vi "demo_proj.vi"() -> ()   [LabVIEW 2015]
doc: "该模板用于创建生产者／消费者模式的应用程序，以事件驱动的方式，生成队列中的项。如需通过响应事件实现代码的异步执行，同时不影响用户界面的响应速度，可考虑用该模式替代用户界面事件处理器模式。"
panel:
  in  "设备类型":enum16{"LAN", "USB"}(ring)=enum."USB"
  in  "波形分析":bool
  in  "读取波形":bool
  in  "波形读取模式":enum32{"bin", "csv"}(radio)
  in  "读取的字节数":u32=400
  in  "读数据":bool
  in  "发指令":bool
  in  "指令集合":string(combo)="mea:all?;"
  in  "清空信息":bool
  out "输出信息":string
  in  "关闭设备":bool
  in  "超时时间(ms)":u32=2000
  out "会话ID":i32
  in  "打开设备":bool
  in  "设备集合":string(combo)
  in  "搜索设备":bool caption="元素入队列"
  in  "停止":bool
  out "数据缓存":u8[](array[numeric])
  out "波形图":sgl[](graph)
  out "波形数据":sgl[](array[numeric])
  out "csv文件输出路径":string
  out "data_out":sgl[](array[numeric])
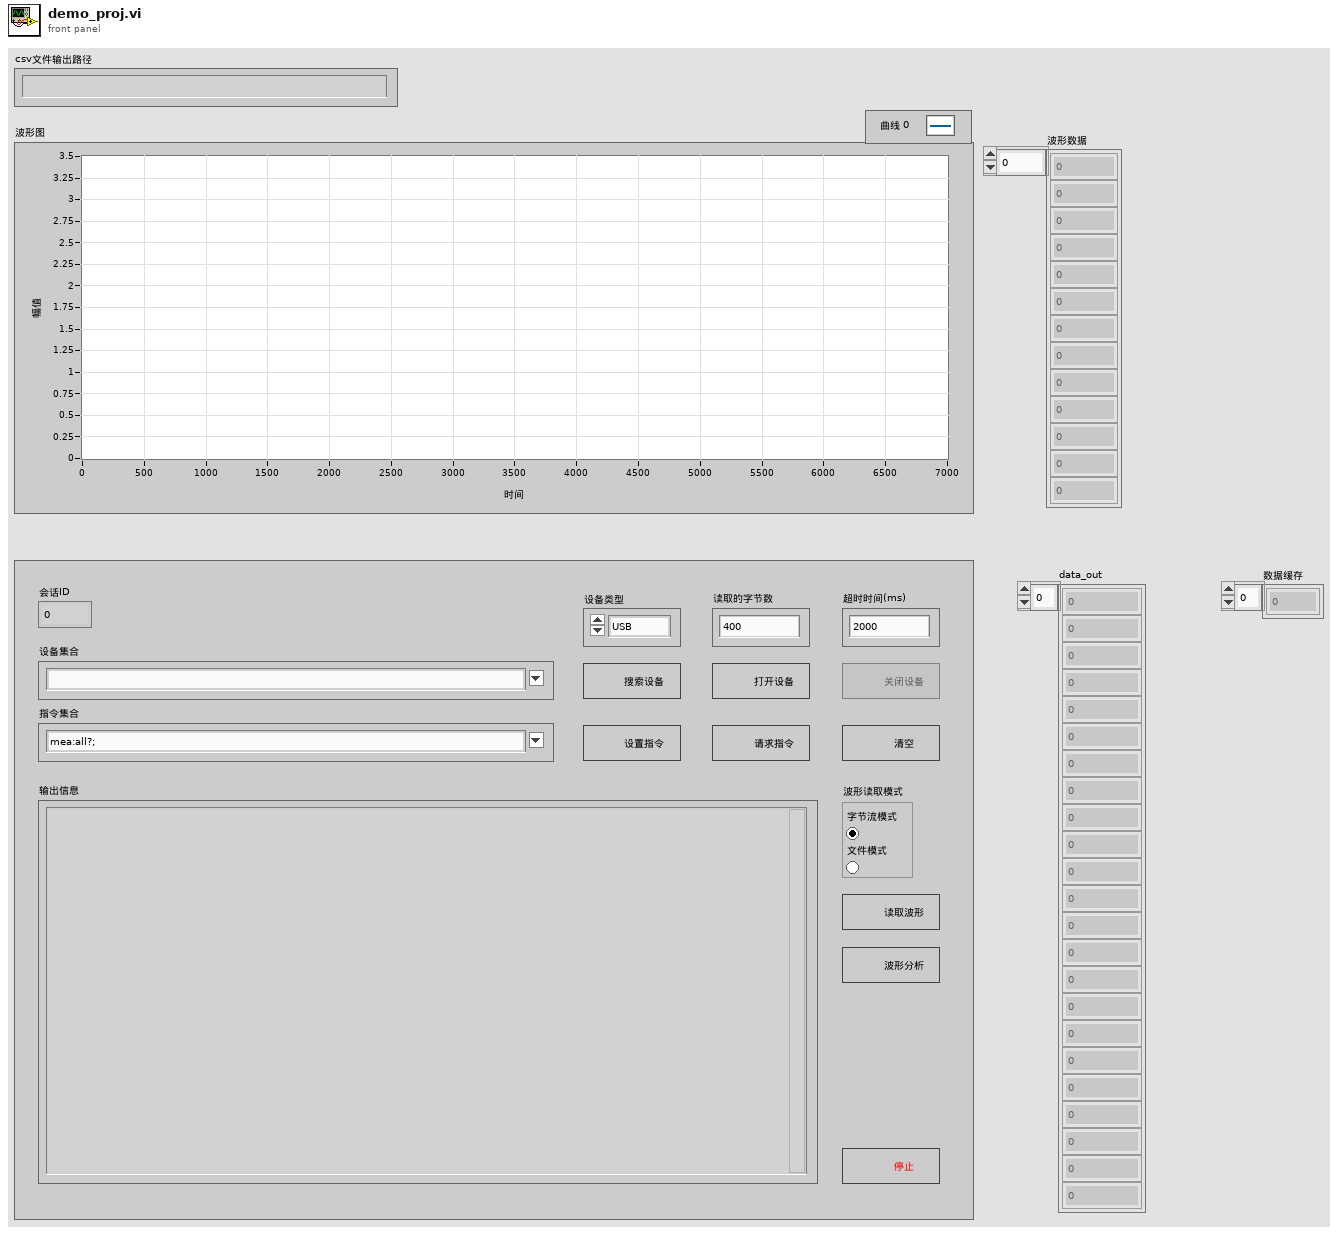
[diagram p1: front panel]
types:
  T1 = enum8{"Enabled", "Disabled", "Disabled and Grayed Out"}
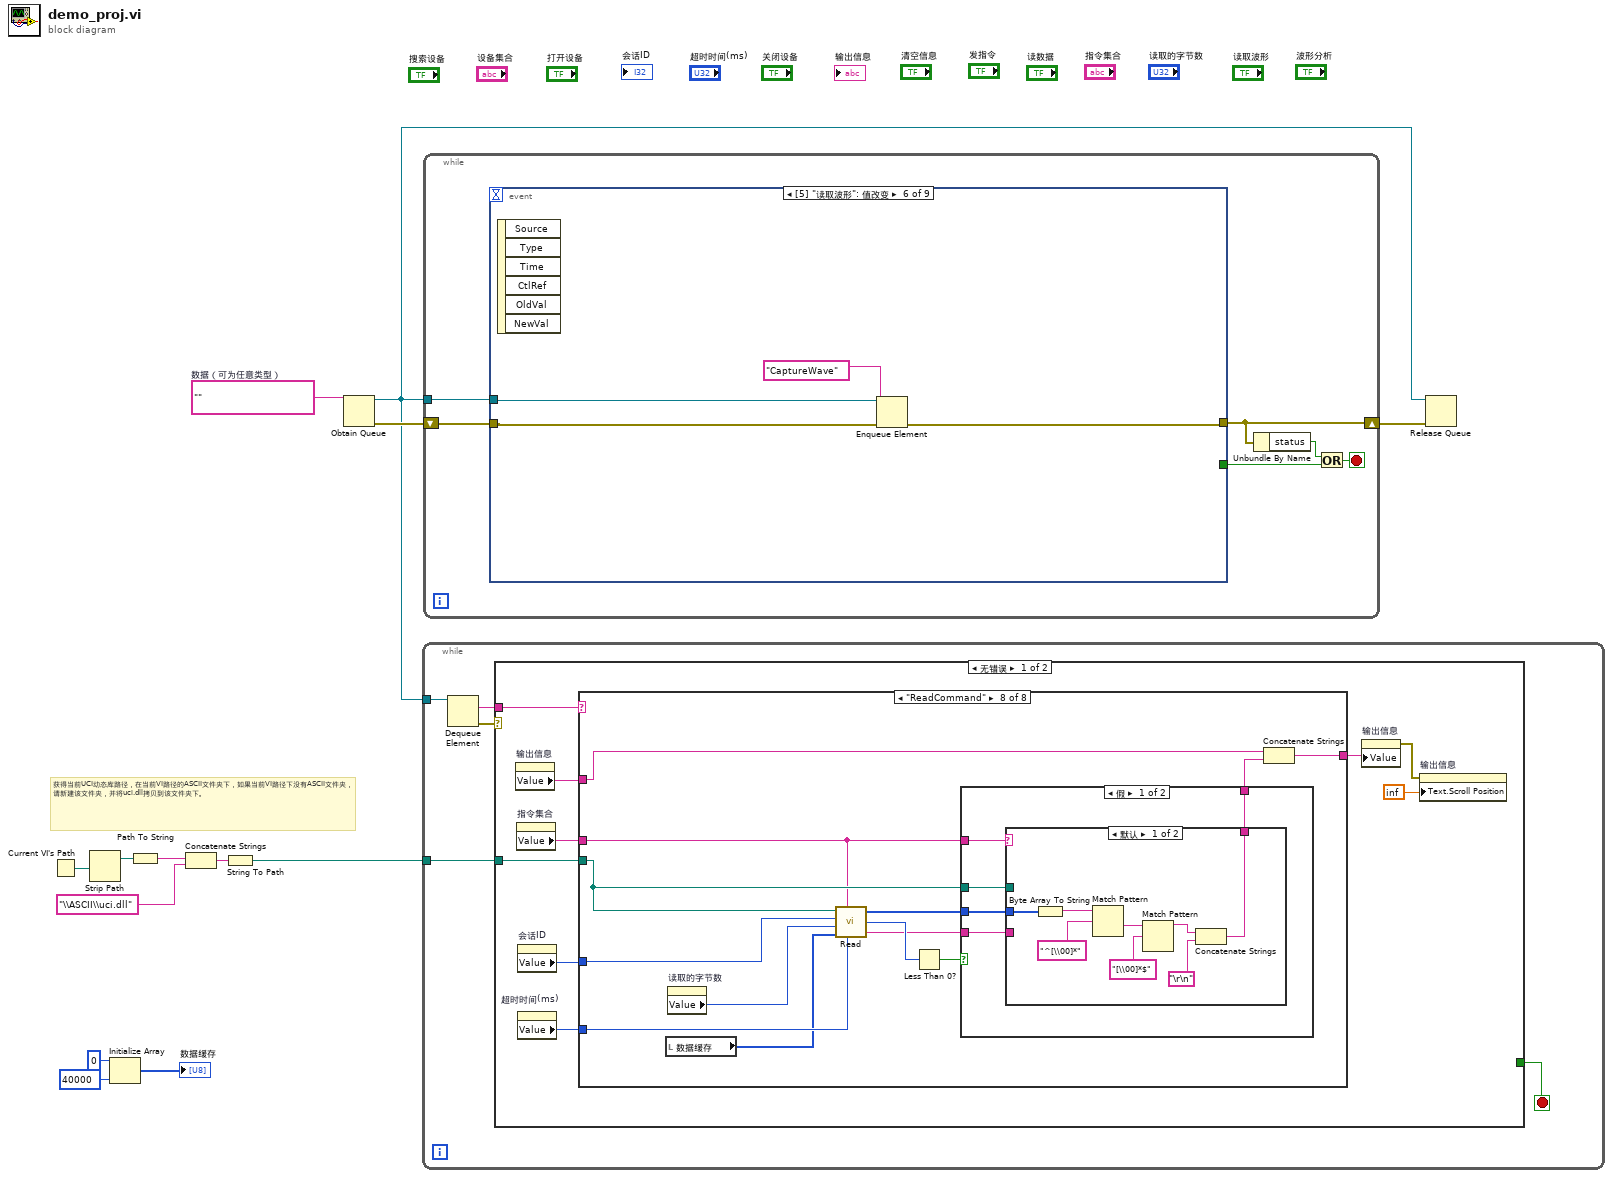
[diagram p0: block diagram]
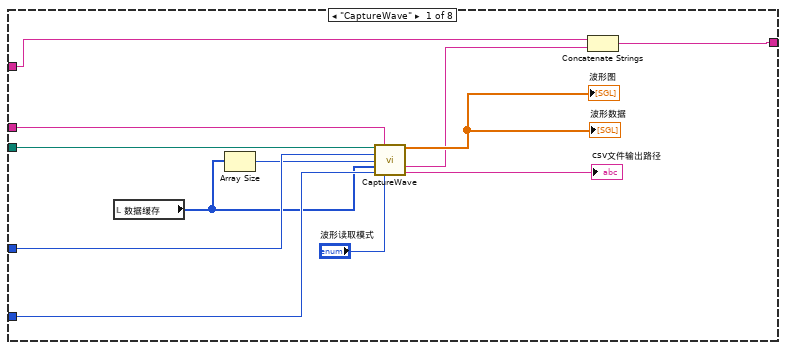
[diagram p2: hidden frame]
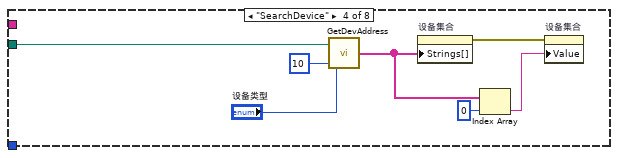
[diagram p5: hidden frame]
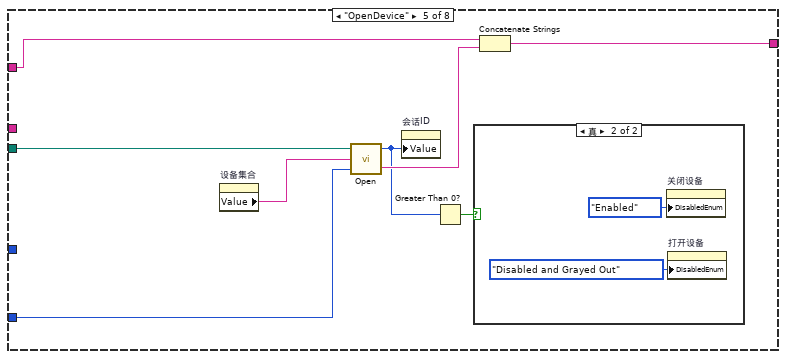
[diagram p6: hidden frame]
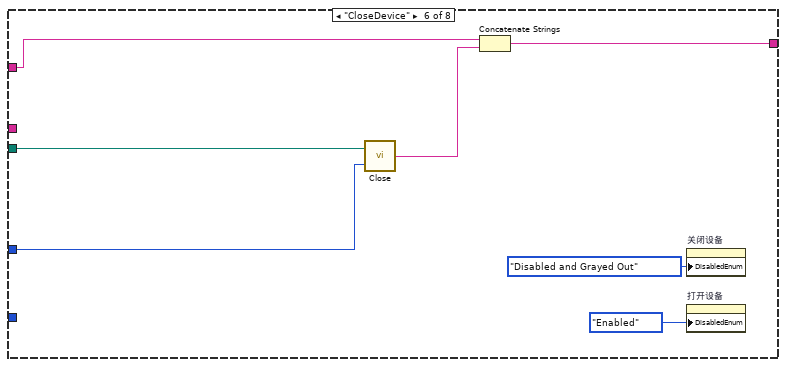
[diagram p8: hidden frame]
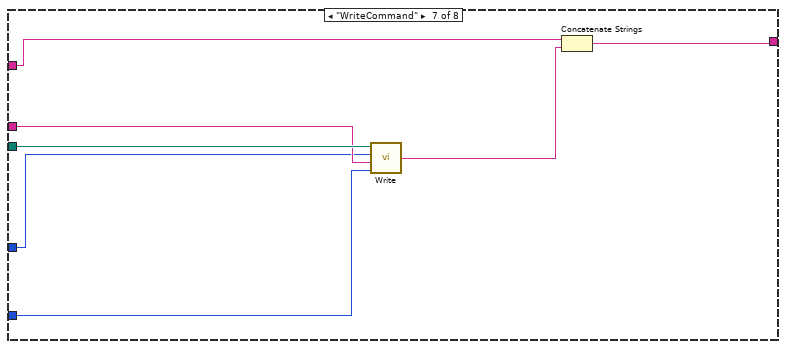
[diagram p9: hidden frame]
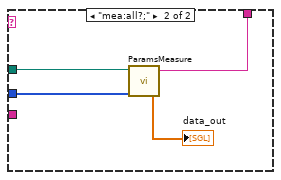
[diagram p10: hidden frame]
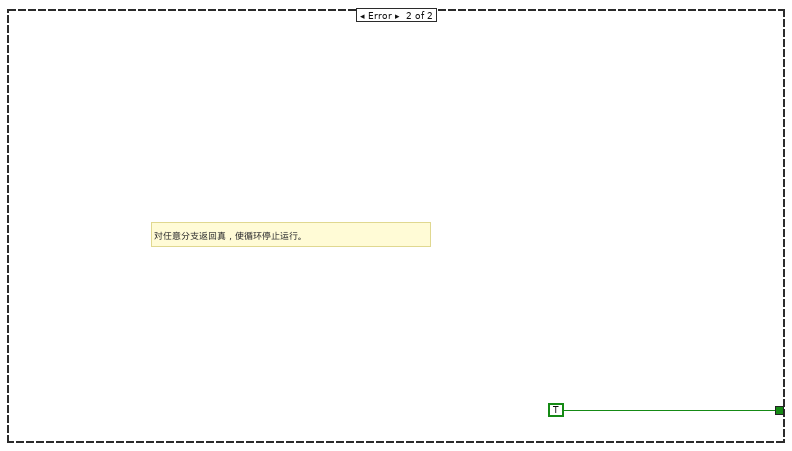
[diagram p12: hidden frame]
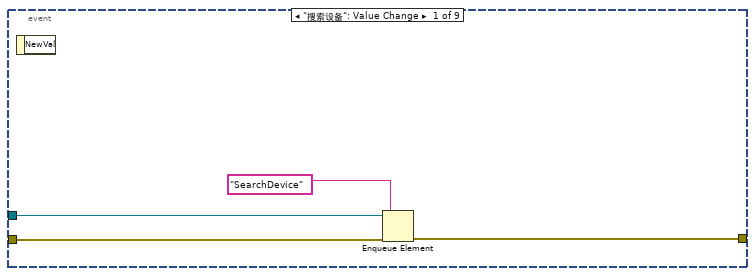
[diagram p13: hidden frame]
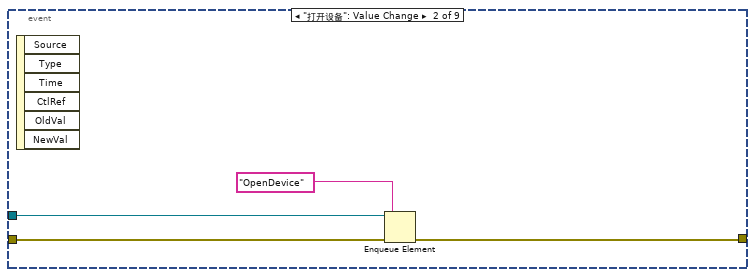
[diagram p14: hidden frame]
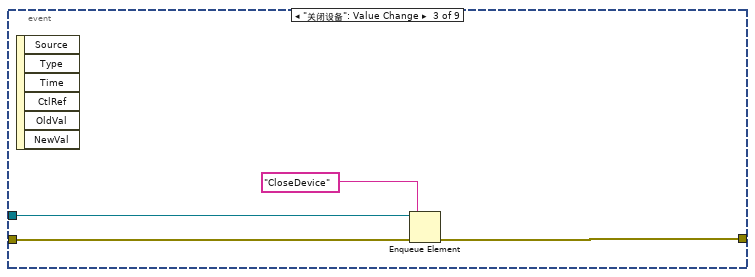
[diagram p15: hidden frame]
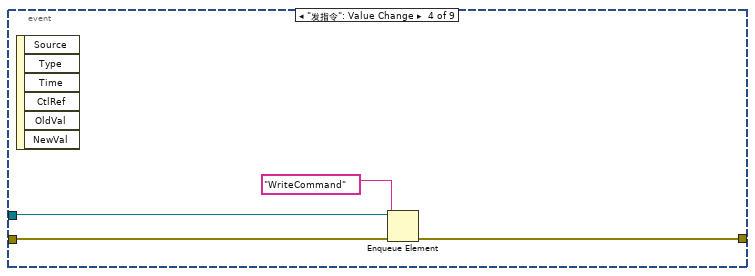
[diagram p16: hidden frame]
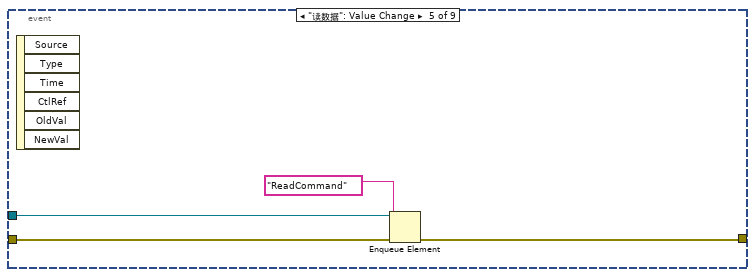
[diagram p17: hidden frame]
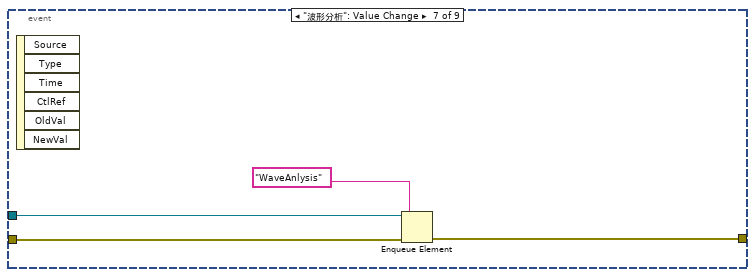
[diagram p18: hidden frame]
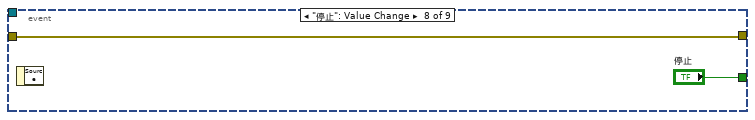
[diagram p19: hidden frame]
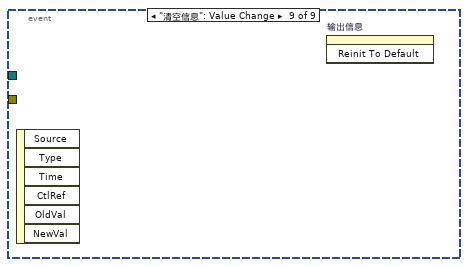
[diagram p20: hidden frame]
diagram:
  w11 = ""  # 数据（可为任意类型）
  # "获得当前UCI动态库路径，在当前VI路径的ASCII文件夹下，如果当前VI路径下没有ASCII文件夹，请新建该文件夹，并将uci.dll拷贝到该文件夹下。"
  n1 = Current VI's Path() -> (path=w8:path)
  n2 = Strip Path(path=w8) -> (stripped path=w6:path)  [unwired: 1 out]
  n3 = Initialize Array(u8 0 ("元素"), 40000 ("维数大小")) -> (→"数据缓存":u8[])
  n4 = Path To String(path=w6) -> (string=w5:string)
  n5 = Concatenate Strings(w5, "\\ASCII\\uci.dll" ("字符串")) -> (w7:string)
  n6 = String To Path(string=w7) -> (path=w4:path)
  n7 = Obtain Queue(element data type=w11) -> (queue out=w10:refnum<queue>, error out=w13:errorcluster)  [unwired: 4 in, 1 out]
  n8 = while {
    tunnel: w10 -> [w18]
    tunnel: w4 -> [w14]
    stop <- w15 stop-if-true
    n9 = Dequeue Element(queue=w18) -> (element=w16:string, error out=w17:errorcluster)  [unwired: 2 in, 2 out]
    n10 = case shown="无错误" w17 {
      tunnel: w16 -> [w27 _]
      tunnel: [_ TRUE] -> w15
      tunnel: w14 -> [w26 _]
      frame No Error {
        n11 = property on="输出信息" class="Str"() -> ("Value"=w25:string)  [unwired: 2 in, 2 out]
        n12 = property on="指令集合" class="CmbBox"() -> ("Value"=w24:string)  [unwired: 2 in, 2 out]
        n13 = property on="会话ID" class="DigNum (严格)"() -> ("Value"=w23:i32)  [unwired: 2 in, 2 out]
        n14 = property on="超时时间(ms)" class="DigNum (严格)"() -> ("Value"=w22:u32)  [unwired: 2 in, 2 out]
        n15 = case shown="\"ReadCommand\"" w27 {
          tunnel: w26 -> [w39 _ _ w46 w54 w63 w70 w82]
          tunnel: w24 -> [w36 _ _ _ _ _ w69 w76]
          tunnel: w23 -> [w38 _ _ _ _ w61 w68 w75]
          tunnel: w25 -> [w30 _ _ _ w50 w59 w64 w74]
          tunnel: [w31 _ _ _ w49 w60 w65 w73] -> w21
          tunnel: w22 -> [w37 _ _ _ w51 _ w67 w72]
          frame "CaptureWave" {
            n16 = local read "数据缓存"() -> (w28:u8[])
            n17 = Array Size(array=w28) -> (size(s)=w29:i32)
            n18 = call "CaptureWave.vi"("UCI_DllPath"=w39, "Command"=w36, "Session_id"=w38, "Length"=w29, "InputData"=w28, "Timeout(ms)"=w37, "ReadType"="波形读取模式") -> ("OutputData"=→"波形数据" →"波形图":sgl[], "ResultDescription"=w32:string, ".csv File Path"=→"csv文件输出路径":string)  [unwired: 6 in]
            n19 = Concatenate Strings(w30, w32) -> (w31:string)
          }
          frame "WaveAnlysis" {
          }
          frame Default {
          }
          frame "SearchDevice" {
            n20 = call "GetDevAddress.vi"("DevNum"=u32 10 ("设备数量"), "DevType"="设备类型", "UCI_DllPath"=w46) -> ("DevAddressGroup"=w43:string[])
            n21 = property on="设备集合" class="CmbBox"("Strings[]"=w43) -> (error out=w44:errorcluster)  [unwired: 2 in, 1 out]
            n22 = Index Array(array=w43, index=0 ("索引")) -> (element=w41:string)
            n23 = property on="设备集合" class="CmbBox"(error in=w44, "Value"=w41) -> ()  [unwired: 1 in, 2 out]
          }
          frame "OpenDevice" {
            n24 = property on="设备集合" class="CmbBox"() -> ("Value"=w53:string)  [unwired: 2 in, 2 out]
            n25 = call "Open.vi"("Timeout"=w51, "Addr"=w53, "UCI_DllPath"=w54) -> ("ResultDescription"=w52:string, "Session_id"=w48:i32)  [unwired: 1 out]
            n26 = property on="会话ID" class="DigNum (严格)"("Value"=w48) -> ()  [unwired: 2 in, 2 out]
            n27 = Greater Than 0?(x=w48) -> (x > 0?=w47:bool)
            n28 = case shown="真" w47 {
              frame False {
              }
              frame True {
                n29 = property on="关闭设备" class="Bool"("DisabledEnum"=T1."Enabled" ("禁用")) -> ()  [unwired: 2 in, 2 out]
                n30 = property on="打开设备" class="Bool"("DisabledEnum"=T1."Disabled and Grayed Out" ("禁用")) -> ()  [unwired: 2 in, 2 out]
              }
            }
            n31 = Concatenate Strings(w50, w52) -> (w49:string)
          }
          frame "CloseDevice" {
            n32 = call "Close.vi"("Session_id"=w61, "UCI_DllPath"=w63) -> ("ResultDescription"=w62:string)
            n33 = Concatenate Strings(w59, w62) -> (w60:string)
            n34 = property on="关闭设备" class="Bool"("DisabledEnum"=T1."Disabled and Grayed Out" ("禁用")) -> ()  [unwired: 2 in, 2 out]
            n35 = property on="打开设备" class="Bool"("DisabledEnum"=T1."Enabled" ("禁用")) -> ()  [unwired: 2 in, 2 out]
          }
          frame "WriteCommand" {
            n36 = call "Write.vi"("UCI_DllPath"=w70, "Session_id"=w68, "Command"=w69, "Timeout"=w67) -> ("ResultDescription"=w66:string)  [unwired: 1 in]
            n37 = Concatenate Strings(w64, w66) -> (w65:string)
          }
          frame "ReadCommand" {
            n38 = local read "数据缓存"() -> (w71:u8[])
            n39 = property on="读取的字节数" class="DigNum (严格)"() -> ("Value"=w81:u32)  [unwired: 2 in, 2 out]
            n40 = call "Read.vi"("UCI_DllPath"=w82, "Command"=w76, "Session_id"=w75, "Length"=w81, "Timeout"=w72, "InputData"=w71) -> ("OutputData"=w83:u8[], "Result"=w79:i32, "ResultDescription"=w77:string)
            n41 = Less Than 0?(x=w79) -> (x < 0?=w78:bool)
            n42 = case shown="假" w78 {
              tunnel: w83 -> [w88 _]
              tunnel: w82 -> [w87 _]
              tunnel: [w86 w101] -> w80
              tunnel: w77 -> [w84 w101]
              tunnel: w76 -> [w85 _]
              frame False {
                n43 = case shown="默认" w85 {
                  tunnel: w88 -> [w93 w100]
                  tunnel: w87 -> [_ w98]
                  tunnel: [w90 w97] -> w86
                  tunnel: w84 -> [_ _]
                  frame Default {
                    n44 = Byte Array To String(unsigned byte array=w93) -> (string=w92:string)
                    n45 = Match Pattern(string=w92, regular expression="^[\\00]*") -> (after substring=w96:string)  [unwired: 1 in, 3 out]
                    n46 = Match Pattern(string=w96, regular expression="[\\00]*$") -> (before substring=w89:string)  [unwired: 1 in, 3 out]
                    n47 = Concatenate Strings(w89, "\r\n") -> (w90:string)
                  }
                  frame "mea:all?;" {
                    n48 = call "ParamsMeasure.vi"("InputData"=w100, "UCI_DllPath"=w98) -> ("OuputData"=→"data_out":sgl[], "OutputString"=w97:string)  [unwired: 3 in]
                  }
                }
              }
              frame True {
              }
            }
            n49 = Concatenate Strings(w74, w80) -> (w73:string)
          }
        }
        n50 = property on="输出信息" class="Str"("Value"=w21) -> (error out=w19:errorcluster)  [unwired: 2 in, 1 out]
        n51 = property on="输出信息" class="Str"(error in=w19, "Text.Scroll Position"=inf) -> ()  [unwired: 1 in, 2 out]
      }
      frame Error {
        # "对任意分支返回真，使循环停止运行。"
      }
    }
  }
  n52 = while {
    shift-right: [w104] -> w12
    shift-left: w13 -> [w107]
    tunnel: w10 -> [w108]
    stop <- w105 stop-if-true
    n53 = event shown="[5] \"读取波形\": 值改变" {
      selector: _ -> [_ _ _ _ _ _ _ _ _]
      dyn-events: _ -> [_ _ _ _ _ _ _ _ _]
      timeout: _ -> [_ _ _ _ _ _ _ _ _]
      tunnel: w108 -> [w112 w115 w119 w123 w127 w131 w135 _ _]
      tunnel: w107 -> [w111 w114 w118 w122 w126 w130 w134 w137 _]
      tunnel: [w110 w113 w117 w124 w125 w129 w133 w137 _] -> w104
      tunnel: [_ _ _ _ _ _ _ "停止" _] -> w106
      event "搜索设备": Value Change {
        n54 = event-data() -> ()  [unwired: 1 in, 1 out]
        n55 = Enqueue Element(queue=w112, element="SearchDevice", error in (no error)=w111) -> (error out=w110:errorcluster)  [unwired: 1 in, 2 out]
      }
      event "打开设备": Value Change {
        n56 = event-data() -> ()  [unwired: 1 in, 6 out]
        n57 = Enqueue Element(queue=w115, element="OpenDevice", error in (no error)=w114) -> (error out=w113:errorcluster)  [unwired: 1 in, 2 out]
      }
      event "关闭设备": Value Change {
        n58 = event-data() -> ()  [unwired: 1 in, 6 out]
        n59 = Enqueue Element(queue=w119, element="CloseDevice", error in (no error)=w118) -> (error out=w117:errorcluster)  [unwired: 1 in, 2 out]
      }
      event "发指令": Value Change {
        n60 = event-data() -> ()  [unwired: 1 in, 6 out]
        n61 = Enqueue Element(queue=w123, element="WriteCommand", error in (no error)=w122) -> (error out=w124:errorcluster)  [unwired: 1 in, 2 out]
      }
      event "读数据": Value Change {
        n62 = event-data() -> ()  [unwired: 1 in, 6 out]
        n63 = Enqueue Element(queue=w127, element="ReadCommand", error in (no error)=w126) -> (error out=w125:errorcluster)  [unwired: 1 in, 2 out]
      }
      event "读取波形": Value Change {
        n64 = event-data() -> ()  [unwired: 1 in, 6 out]
        n65 = Enqueue Element(queue=w131, element="CaptureWave", error in (no error)=w130) -> (error out=w129:errorcluster)  [unwired: 1 in, 2 out]
      }
      event "波形分析": Value Change {
        n66 = event-data() -> ()  [unwired: 1 in, 6 out]
        n67 = Enqueue Element(queue=w135, element="WaveAnlysis", error in (no error)=w134) -> (error out=w133:errorcluster)  [unwired: 1 in, 2 out]
      }
      event "停止": Value Change {
        n68 = event-data() -> ()  [unwired: 1 in, 1 out]
      }
      event "清空信息": Value Change {
        n69 = event-data() -> ()  [unwired: 1 in, 6 out]
        n70 = invoke on="输出信息" class="Str" method="Reinit To Default"() -> ()  [unwired: 3 in, 3 out]
      }
    }
    n71 = Unbundle By Name(w104) -> ("status"=w103:bool)
    n72 = Or(x=w103, y=w106) -> (x .or. y?=w105:bool)
  }
  n73 = Release Queue(queue=w10, error in (no error)=w12) -> ()  [unwired: 1 in, 3 out]
